vi "PIDController_AdvExecute.vi"(0 "Time":dbl=-1.0 format="%33.4f", 4 "Reset":bool, 5 "PID Error Tolerance":T2={"PositionTolerance"=0.001, "VelocityTolerance"=9.9e+30}, 6 "Auto":bool=TRUE, 7 "Adv PID Limits":T1={"MaxInput"=0.0, "MinInput"=0.0, "Continuous"=FALSE, "MaxOutput"=9.9e+32, "MinOutput"=-9.9e+32}, 8 "FF-FeedForward":dbl, 9 "SP-SetPoint":dbl, 10 "PV-Measurement":dbl, 11 "Adv PID Tuning":T3={"Kf"=0.0, "Kp"=0.0, "Ki"=0.0, "Kd"=0.0, "MaximumIntegral"=9.9e+30, "MinimumIntegral"=-9.9e+30, "Filter Derivative"=FALSE, "IntegralZone"=9.9e+30}) -> (1 "AtSetpoint":bool, 2 "CO-ControlOutput":dbl, 3 "out PID_CONTROLLER":T4={"Kp"=0.0, "Ki"=0.0, "Kd"=0.0, "Period"=0.0, "Max_Integral"=0.0, "Min_Integral"=0.0, "Max_Input"=0.0, "Min_Input"=0.0, "Continuous"=FALSE, "PositionError"=0.0, "VelocityError"=0.0, "PrevError"=0.0, "Total_Integral"=0.0, "PositionTolerance"=0.0, "VelocityTolerance"=0.0, "SetPoint"=0.0, "Kf"=0.0, "Prev_Deriv"=0.0, "Prev_Deriv 2"=0.0, "DerivativeFilter"=FALSE, "Min_Output"=-9.99e+35, "Max_Output"=9.9e+35, "Prev_F_P"=0.0, "Prev_F_P_2"=0.0, "AntiWindupActive"=FALSE, "Measurement"=0.0, "IntegralZone"=9.9e+30} {"IntegralZone" format="%16_6e"; "Measurement" format="%16_6e"; "Prev_F_P_2" format="%16_6e"; "Prev_F_P" format="%16_6e"; "Max_Output" format="%16_6e"; "Min_Output" format="%16_6e"; "Prev_Deriv 2" format="%16_6e"; "Prev_Deriv" format="%16_6e"; "Kf" format="%16_6e"; "SetPoint" format="%16_6e"; "VelocityTolerance" format="%16_6e"; "PositionTolerance" format="%16_6e"; "Total_Integral" format="%16_6e"; "PrevError" format="%16_6e"; "VelocityError" format="%16_6e"; "PositionError" format="%16_6e"; "Min_Input" format="%16_6e"; "Max_Input" format="%16_6e"; "Min_Integral" format="%16_6e"; "Max_Integral" format="%16_6e"; "Period" format="%16_6e"; "Kd" format="%16_6e"; "Ki" format="%16_6e"; "Kp" format="%16_6e"})   [LabVIEW 2019, in "Trajectory_Library.lvlib"]
doc: "Convience, single call, LabVIEW function. Creates and calculates the \"advanced\" PID controller. Call this routine periodically to calculate the newest output for the provided inputs. \n\nSee the \"PID Adv Calculate\" VI documentation for additional details on the \"advanced PID\"\n \nInputs:\n - PID Error Tolerance -- Tolerances for determining \"At Setpoint\", contains:\n - Position Tolerance -- (Default: 0.001)\n - Velocity Tolerance -- (Default: 9.9E+30)\n - Adv PID Limits -- Cluster containing:\n - MaxInput -- (Default: 0)\n - MinInput -- (Default: 0)\n - Continous -- When True indicates that the input is continuous. (Default: False)\n - MaxOutput -- The largest allowed value for the control output (CO) \n - MinOutput -- The smallest allowed value for the control output (CO)\n - PID Tuning -- PID Tuning parameters containing:\n - Kf -- The feedforward gain coefficient.\n - Kp -- The proportional coefficient.\n - Ki -- The integral coefficient.\n - Kd -- The derivative coefficient.\n - Maximum Integral -- The maximum value of the integrator.\n - Minimum Integral -- The minimum value of the integrator.\n - Filter Derivative -- Use derivative filtering when True.\n - PV-measurement -- The current measurement of the process variable. (PV)\n - SP-setpoint -- The new setpoint of the controller. (SP)\n - FF-Feedforward -- The feedforward value. \n - Auto -- Use the PID calculate when this is True\n - Reset -- When True, causes the PID to be reset. (Default: False)\n\nOutputs:\n - PID_Controller -- Updated PID_Controller data cluster\n - CO-ControlOutput -- Controller output (CO) \n - AtSetpoint -- True when PV is within the specified tolerances of the SP."
uses:
  Trajectory_Library.lvlib
  TypeDef/PID_CONTROLLER.ctl
  TypeDef/PID_ADV_TUNING.ctl
  TypeDef/PID_ERROR_TOLERANCE.ctl
  TypeDef/PID_ADV_LIMITS.ctl
  PIDController_NewPeriod.vi
  <vilib>/Rock Robotics/SystemInterfaces/NetworkCommunication/NetComm_UsageReport_report.vi
  Globals/Util_LibraryGlobals.vi
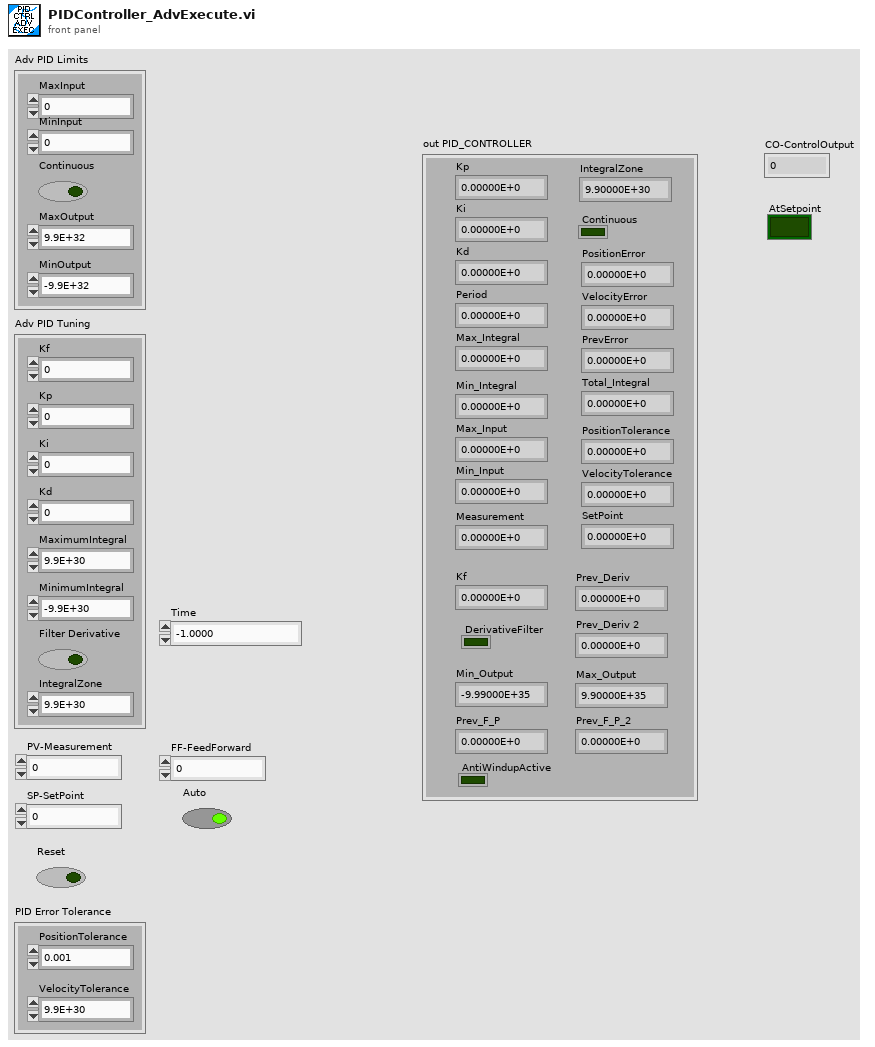
[diagram p1: front panel]
types:
  T1 = typedef "Trajectory_Library.lvlib/PID_ADV_LIMITS.ctl" = cluster{"MaxInput":dbl, "MinInput":dbl, "Continuous":bool, "MaxOutput":dbl, "MinOutput":dbl}
  T2 = typedef "Trajectory_Library.lvlib/PID_ERROR_TOLERANCE.ctl" = cluster{"PositionTolerance":dbl, "VelocityTolerance":dbl}
  T3 = typedef "Trajectory_Library.lvlib/PID_ADV_TUNING.ctl" = cluster{"Kf":dbl, "Kp":dbl, "Ki":dbl, "Kd":dbl, "MaximumIntegral":dbl, "MinimumIntegral":dbl, "Filter Derivative":bool, "IntegralZone":dbl}
  T4 = typedef "Trajectory_Library.lvlib/PID_CONTROLLER.ctl" = cluster{"Kp":dbl, "Ki":dbl, "Kd":dbl, "Period":dbl, "Max_Integral":dbl, "Min_Integral":dbl, "Max_Input":dbl, "Min_Input":dbl, "Continuous":bool, "PositionError":dbl, "VelocityError":dbl, "PrevError":dbl, "Total_Integral":dbl, "PositionTolerance":dbl, "VelocityTolerance":dbl, "SetPoint":dbl, "Kf":dbl, "Prev_Deriv":dbl, "Prev_Deriv 2":dbl, "DerivativeFilter":bool, "Min_Output":dbl, "Max_Output":dbl, "Prev_F_P":dbl, "Prev_F_P_2":dbl, "AntiWindupActive":bool, "Measurement":dbl, "IntegralZone":dbl}
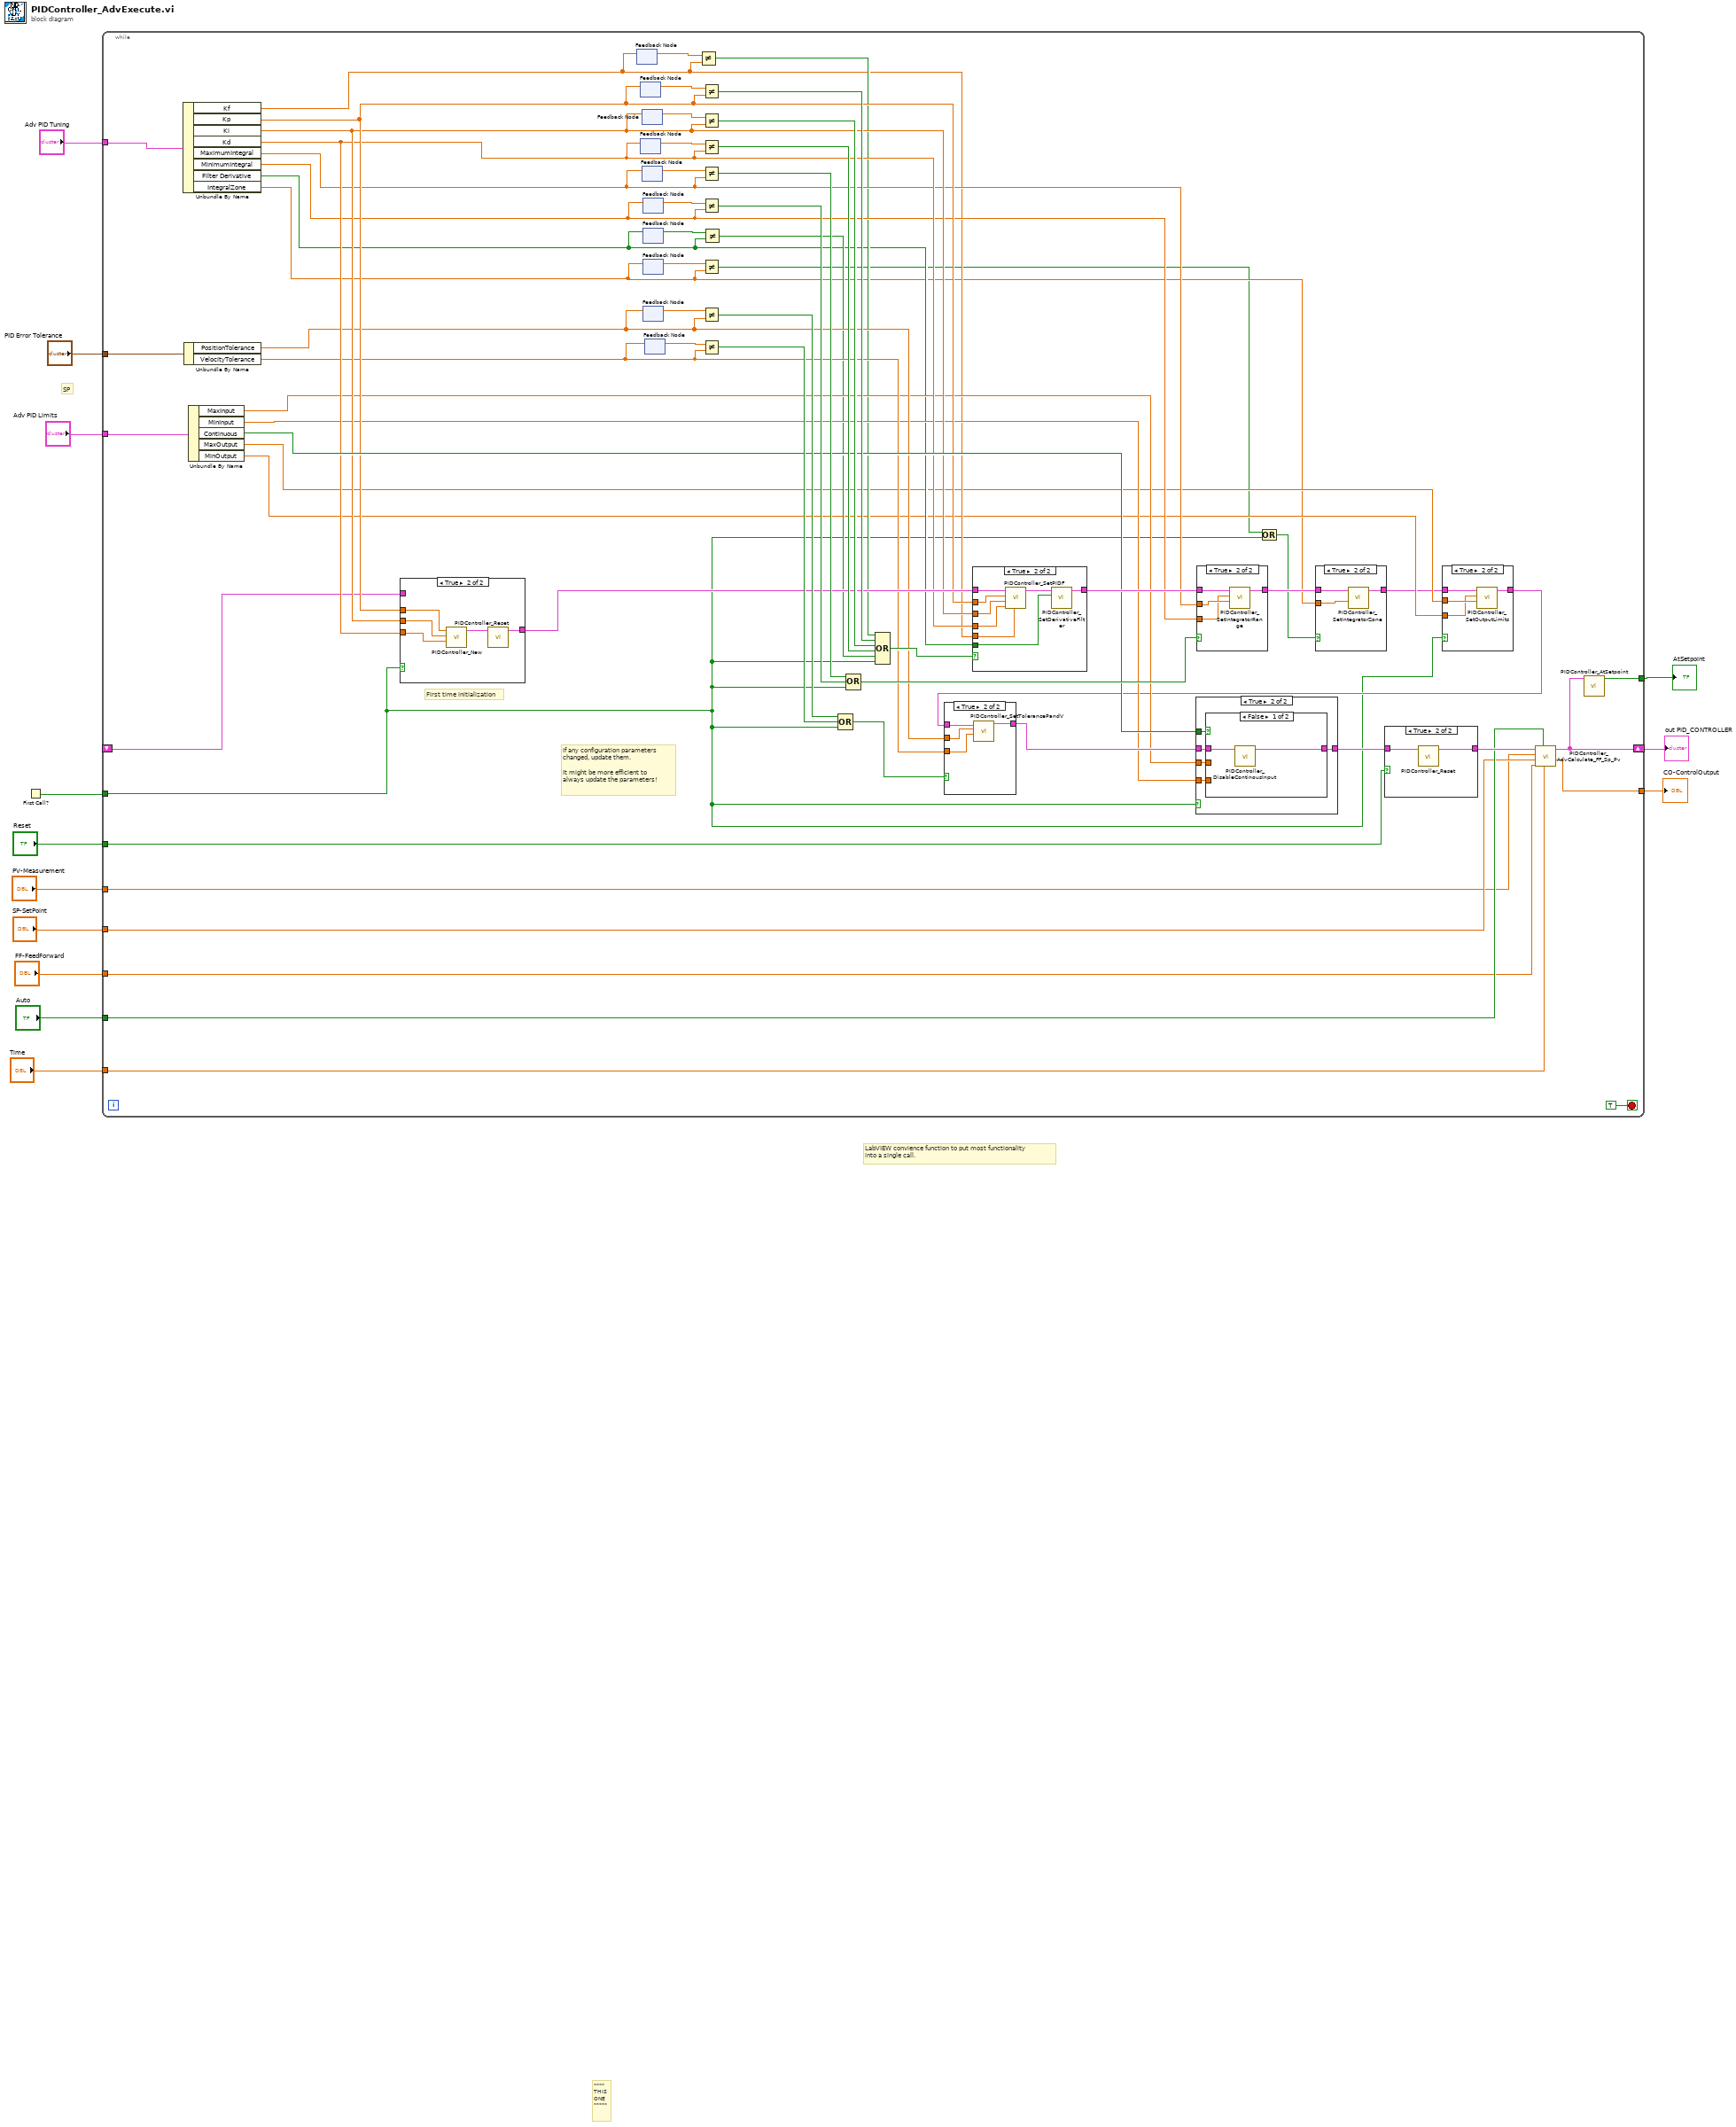
[diagram p0: block diagram]
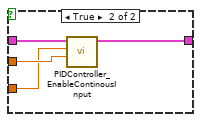
[diagram p7: hidden frame]
diagram:
  # "SP"
  # "LabVIEW convience function to put most functionality\ninto a single call."
  # "****\nTHIS\nONE\n*****"
  n1 = First Call?() -> (First Call?: T/F=w1:bool)
  n2 = while {
    tunnel: "Adv PID Tuning" -> [w75]
    tunnel: [w74] -> w12
    tunnel: "PID Error Tolerance" -> [w73]
    tunnel: "Adv PID Limits" -> [w72]
    tunnel: [w39] -> w8
    tunnel: "Time" -> [w27]
    tunnel: "Auto" -> [w26]
    tunnel: "FF-FeedForward" -> [w25]
    tunnel: "Reset" -> [w24]
    tunnel: "SP-SetPoint" -> [w23]
    tunnel: "PV-Measurement" -> [w22]
    shift-right: [w40] -> w9
    shift-left: _ -> [w21]
    tunnel: w1 -> [w14]
    stop <- TRUE stop-if-true
    # "First time initialization"
    # "If any configuration parameters \nchanged, update them.\n\nIt might be more efficient to\nalways update the parameters!"
    n3 = Unbundle By Name(w75) -> ("Kf"=w35:dbl, "Kp"=w56:dbl, "Ki"=w55:dbl, "Kd"=w54:dbl, "MaximumIntegral"=w53:dbl, "MinimumIntegral"=w52:dbl, "Filter Derivative"=w32:bool, "IntegralZone"=w17:dbl)
    n4 = Unbundle By Name(w73) -> ("PositionTolerance"=w51:dbl, "VelocityTolerance"=w50:dbl)
    n5 = Unbundle By Name(w72) -> ("MaxInput"=w49:dbl, "MinInput"=w48:dbl, "Continuous"=w57:bool, "MaxOutput"=w30:dbl, "MinOutput"=w29:dbl)
    n6 = case shown="True" w14 {
      tunnel: w56 -> [_ w88]
      tunnel: w55 -> [_ w87]
      tunnel: w54 -> [_ w86]
      tunnel: [w85 w90] -> w58
      tunnel: w21 -> [w85 _]
      frame False {
      }
      frame True {
        n7 = call "PIDController_New.vi"("Kd"=w86, "Ki"=w87, "Kp"=w88) -> ("PID_CONTROLLER"=w89:T4)  [unwired: 8 in]
        n8 = call "PIDController_Reset.vi"("in PID_CONTROLLER"=w89) -> ("out PID_CONTROLLER"=w90:T4)  [unwired: 10 in]
      }
    }
    n9 = feedback #1() -> (w37:dbl)  [unwired: 1 in]
    n10 = feedback-in #1(w35) -> ()
    n11 = feedback #2() -> (w47:dbl)  [unwired: 1 in]
    n12 = feedback-in #2(w56) -> ()
    n13 = feedback #3() -> (w45:dbl)  [unwired: 1 in]
    n14 = feedback-in #3(w54) -> ()
    n15 = feedback #4() -> (w46:dbl)  [unwired: 1 in]
    n16 = feedback-in #4(w55) -> ()
    n17 = feedback #5() -> (w44:dbl)  [unwired: 1 in]
    n18 = feedback-in #5(w53) -> ()
    n19 = feedback #6() -> (w43:dbl)  [unwired: 1 in]
    n20 = feedback-in #6(w52) -> ()
    n21 = feedback #7() -> (w20:dbl)  [unwired: 1 in]
    n22 = feedback-in #7(w17) -> ()
    n23 = feedback #8() -> (w42:dbl)  [unwired: 1 in]
    n24 = feedback-in #8(w51) -> ()
    n25 = feedback #9() -> (w34:bool)  [unwired: 1 in]
    n26 = feedback-in #9(w32) -> ()
    n27 = feedback #10() -> (w41:dbl)  [unwired: 1 in]
    n28 = feedback-in #10(w50) -> ()
    n29 = Not Equal?(x=w37, y=w35) -> (x != y?=w36:bool)
    n30 = Not Equal?(x=w47, y=w56) -> (x != y?=w65:bool)
    n31 = Not Equal?(x=w46, y=w55) -> (x != y?=w66:bool)
    n32 = Not Equal?(x=w45, y=w54) -> (x != y?=w67:bool)
    n33 = Not Equal?(x=w44, y=w53) -> (x != y?=w68:bool)
    n34 = Not Equal?(x=w43, y=w52) -> (x != y?=w69:bool)
    n35 = Not Equal?(x=w20, y=w17) -> (x != y?=w15:bool)
    n36 = Not Equal?(x=w42, y=w51) -> (x != y?=w70:bool)
    n37 = Not Equal?(x=w41, y=w50) -> (x != y?=w71:bool)
    n38 = Not Equal?(x=w34, y=w32) -> (x != y?=w33:bool)
    n39 = Compound Arithmetic op=OR(w70, w71, w14) -> (w61:bool)
    n40 = Compound Arithmetic op=OR(w68, w69, w14) -> (w62:bool)
    n41 = Compound Arithmetic op=OR(w36, w65, w66, w67, w33, w14) -> (w64:bool)
    n42 = case shown="True" w64 {
      tunnel: w58 -> [w116 w124]
      tunnel: w56 -> [_ w123]
      tunnel: w55 -> [_ w122]
      tunnel: w54 -> [_ w121]
      tunnel: [w116 w119] -> w63
      tunnel: w35 -> [_ w120]
      tunnel: w32 -> [_ w117]
      frame False {
      }
      frame True {
        n43 = call "PIDController_SetPIDF.vi"("Kf"=w120, "Kd"=w121, "Ki"=w122, "Kp"=w123, "in PID_CONTROLLER"=w124) -> ("out PID_CONTROLLER"=w118:T4)  [unwired: 6 in]
        n44 = call "PIDController_SetDerivativeFilter.vi"("DerivativeFilter"=w117, "in PID_CONTROLLER"=w118) -> ("out PID_CONTROLLER"=w119:T4)  [unwired: 9 in]
      }
    }
    n45 = case shown="True" w62 {
      tunnel: w63 -> [w111 w115]
      tunnel: w53 -> [_ w114]
      tunnel: w52 -> [_ w113]
      tunnel: [w111 w112] -> w19
      frame False {
      }
      frame True {
        n46 = call "PIDController_SetIntegratorRange.vi"("MaximumIntegral"=w114, "MinimumIntegral"=w113, "in PID_CONTROLLER"=w115) -> ("out PID_CONTROLLER"=w112:T4)  [unwired: 8 in]
      }
    }
    n47 = Or(x=w15, y=w14) -> (x .or. y?=w16:bool)
    n48 = case shown="True" w16 {
      tunnel: [w76 w79] -> w18
      tunnel: w19 -> [w76 w78]
      tunnel: w17 -> [_ w77]
      frame False {
      }
      frame True {
        n49 = call "PIDController_SetIntegratorZone.vi"("IntegratorZone"=w77, "in PID_CONTROLLER"=w78) -> ("out PID_CONTROLLER"=w79:T4)  [unwired: 9 in]
      }
    }
    n50 = case shown="True" w14 {
      tunnel: w18 -> [w80 w84]
      tunnel: [w80 w83] -> w31
      tunnel: w30 -> [_ w82]
      tunnel: w29 -> [_ w81]
      frame False {
      }
      frame True {
        n51 = call "PIDController_SetOutputLimits.vi"("MaxOutput"=w82, "MinOutput"=w81, "in PID_CONTROLLER"=w84) -> ("out PID_CONTROLLER"=w83:T4)  [unwired: 8 in]
      }
    }
    n52 = case shown="True" w61 {
      tunnel: w31 -> [w106 w110]
      tunnel: w51 -> [_ w109]
      tunnel: w50 -> [_ w108]
      tunnel: [w106 w107] -> w60
      frame False {
      }
      frame True {
        n53 = call "PIDController_SetTolerancePandV.vi"("VelocityTolerance"=w108, "PositionTolerance"=w109, "in PID_CONTROLLER"=w110) -> ("out PID_CONTROLLER"=w107:T4)  [unwired: 8 in]
      }
    }
    n54 = case shown="True" w14 {
      tunnel: w49 -> [_ w99]
      tunnel: w48 -> [_ w98]
      tunnel: w60 -> [w94 w97]
      tunnel: w57 -> [_ w96]
      tunnel: [w94 w95] -> w59
      frame False {
      }
      frame True {
        n55 = case shown="False" w96 {
          tunnel: w97 -> [w101 w105]
          tunnel: [w100 w104] -> w95
          tunnel: w99 -> [_ w103]
          tunnel: w98 -> [_ w102]
          frame False {
            n56 = call "PIDController_DisableContinousInput.vi"("in PID_CONTROLLER"=w101) -> ("out PID_CONTROLLER"=w100:T4)  [unwired: 10 in]
          }
          frame True {
            n57 = call "PIDController_EnableContinousInput.vi"("MaxInput"=w103, "MinInput"=w102, "in PID_CONTROLLER"=w105) -> ("out PID_CONTROLLER"=w104:T4)  [unwired: 8 in]
          }
        }
      }
    }
    n58 = case shown="True" w24 {
      tunnel: w59 -> [w91 w93]
      tunnel: [w91 w92] -> w38
      frame False {
      }
      frame True {
        n59 = call "PIDController_Reset.vi"("in PID_CONTROLLER"=w93) -> ("out PID_CONTROLLER"=w92:T4)  [unwired: 10 in]
      }
    }
    n60 = call "PIDController_AdvCalculate_FF_Sp_Pv.vi"("Time"=w27, "Auto"=w26, "FF"=w25, "SP"=w23, "PV"=w22, "in PID_CONTROLLER"=w38) -> ("ControlOutput"=w39:dbl, "out PID_CONTROLLER"=w40:T4)  [unwired: 4 in]
    n61 = call "PIDController_AtSetpoint.vi"("in PID_CONTROLLER"=w40) -> ("AtSetpoint"=w74:bool)  [unwired: 10 in]
  }
  "out PID_CONTROLLER" <- w9
  "CO-ControlOutput" <- w8
  "AtSetpoint" <- w12
